vi "Host_Shutdown.vi"(5 "writer ref":refnum<k21>, 6 "reader ref":refnum<k21>, 7 "Queue in":refnum<queue>, 8 "error in 2":errorcluster, 9 "error in 1":errorcluster, 10 "error in 3":errorcluster) -> (2 "error out":errorcluster)   [LabVIEW 2025]
uses:
  vi/Command.ctl
  vi/thresholds.ctl
  vi/RT_Cmd.ctl
  vi/action.ctl
  vi/UI_Msg.ctl
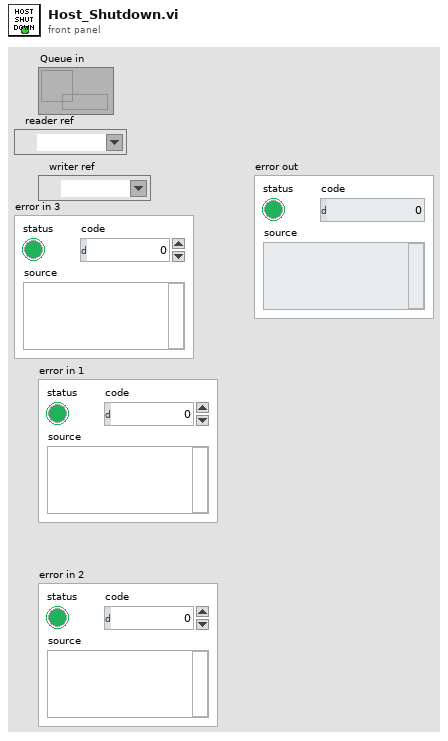
[diagram p1: front panel]
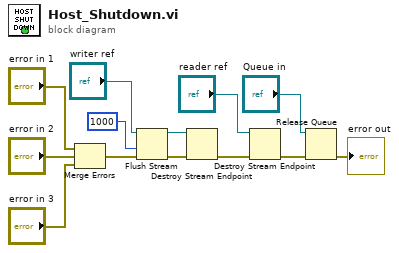
[diagram p0: block diagram]
diagram:
  n1 = Merge Errors("error in 1", "error in 2", "error in 3") -> (w7:errorcluster)
  n2 = Flush Stream(8:w7, 9:1000 ("timeout in ms (-1)"), 11:"writer ref") -> (0:w6:errorcluster, 3:w3:refnum<k21>)  [unwired: 1 in, 1 out]
  n3 = Destroy Stream Endpoint(8:w6, 11:w3) -> (0:w11:errorcluster)
  n4 = Destroy Stream Endpoint(8:w11, 11:"reader ref") -> (0:w2:errorcluster)
  n5 = Release Queue(queue="Queue in", error in (no error)=w2) -> (error out=→"error out":errorcluster)  [unwired: 1 in, 2 out]
